vi "Register gRPC Methods.vi"(8 "error in (no error)":errorcluster, 11 "gRPC service in":refnum<class "CanWriterNixnet.lvclass">) -> (0 "error out":errorcluster, 3 "gRPC service out":refnum<class "CanWriterNixnet.lvclass">)   [LabVIEW 2021, in "CanWriterNixnet_server.lvlib" / "CanWriterNixnet.lvclass"]
uses:
  CanWriterNixnet.lvclass
  typeDefs/Server Internal UEs.ctl
  typeDefs/Server Internal Message.ctl
  typeDefs/Server gRPC UEs.ctl
  <vilib>/gRPC/LabVIEW gRPC Library/Server API/typeDefs/gRPCId Cluster.ctl
  <vilib>/gRPC/LabVIEW gRPC Library/Shared/grpcId.ctl
  CanWriterNixnet.lvclass/CanWriterNixnet.ctl
  <vilib>/gRPC/LabVIEW gRPC Library/grpc-lvsupport-release.lvlib
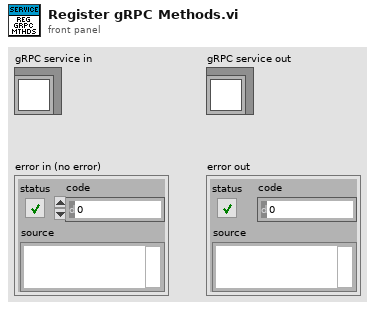
[diagram p1: front panel]
types:
  T1 = typedef "CanWriterNixnet_server.lvlib/CanWriterNixnet.lvclass/Server gRPC UEs.ctl" = cluster{"CanWriterNixnet GetDevices gRPC UE":refnum<user-event>, "CanWriterNixnet GetStatistics gRPC UE":refnum<user-event>, "CanWriterNixnet SetInterfaceBlink gRPC UE":refnum<user-event>, "CanWriterNixnet SendCanMessage gRPC UE":refnum<user-event>, "CanWriterNixnet GetCANStatus gRPC UE":refnum<user-event>}
  T2 = typedef "CanWriterNixnet_server.lvlib/CanWriterNixnet.lvclass/Server Internal UEs.ctl" = cluster{"CanWriterNixnet GetDevices Internal UE":refnum<user-event>, "CanWriterNixnet GetStatistics Internal UE":refnum<user-event>, "CanWriterNixnet SetInterfaceBlink Internal UE":refnum<user-event>, "CanWriterNixnet SendCanMessage Internal UE":refnum<user-event>, "CanWriterNixnet GetCANStatus Internal UE":refnum<user-event>}
  T3 = typedef "grpc-lvsupport-release.lvlib/grpcId.ctl" = u64
  T4 = typedef "CanWriterNixnet_server.lvlib/CanWriterNixnet.lvclass/Server Internal Message UE.ctl" = refnum<user-event>
  T5 = typedef "grpc-lvsupport-release.lvlib/gRPCId Cluster UE.ctl" = refnum<user-event>
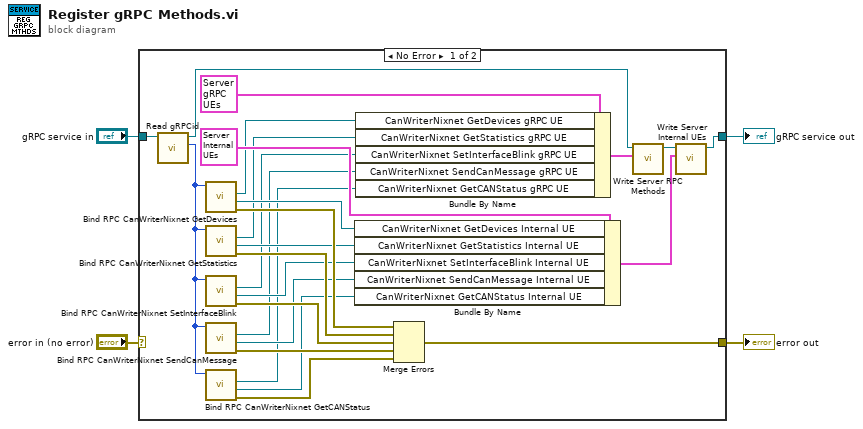
[diagram p0: block diagram]
diagram:
  n1 = case shown="No Error" "error in (no error)" {
    selector: "error in (no error)" -> [_ w30]
    tunnel: "gRPC service in" -> [w21 w31]
    tunnel: [w29 w30] -> w3
    tunnel: [w28 w31] -> w2
    frame No Error {
      n2 = call-dynamic "Read gRPCid.vi"("gRPC service in"=w21) -> ("gRPCid"=w20:T3, "gRPC service out"=w22:refnum<class "CanWriterNixnet.lvclass">)  [unwired: 8 in, 1 out]
      n3 = call "Bind RPC CanWriterNixnet GetDevices.vi"("gRPCid server in"=w20) -> ("error out"=w19:errorcluster, "CanWriterNixnet GetDevices Internal UE"=w17:T4, "CanWriterNixnet GetDevices gRPC UE"=w18:T5)  [unwired: 7 in, 1 out]
      n4 = call "Bind RPC CanWriterNixnet GetStatistics.vi"("gRPCid server in"=w20) -> ("error out"=w16:errorcluster, "CanWriterNixnet GetStatistics Internal UE"=w14:T4, "CanWriterNixnet GetStatistics gRPC UE"=w15:T5)  [unwired: 7 in, 1 out]
      n5 = call "Bind RPC CanWriterNixnet SetInterfaceBlink.vi"("gRPCid server in"=w20) -> ("error out"=w13:errorcluster, "CanWriterNixnet SetInterfaceBlink Internal UE"=w11:T4, "CanWriterNixnet SetInterfaceBlink gRPC UE"=w12:T5)  [unwired: 7 in, 1 out]
      n6 = call "Bind RPC CanWriterNixnet SendCanMessage.vi"("gRPCid server in"=w20) -> ("error out"=w10:errorcluster, "CanWriterNixnet SendCanMessage Internal UE"=w8:T4, "CanWriterNixnet SendCanMessage gRPC UE"=w9:T5)  [unwired: 7 in, 1 out]
      n7 = call "Bind RPC CanWriterNixnet GetCANStatus.vi"("gRPCid server in"=w20) -> ("error out"=w7:errorcluster, "CanWriterNixnet GetCANStatus Internal UE"=w5:T4, "CanWriterNixnet GetCANStatus gRPC UE"=w6:T5)  [unwired: 7 in, 1 out]
      n8 = Bundle By Name ("Bundle Internal UEs")(cluster=T2 {"CanWriterNixnet GetDevices Internal UE"=refnum, "CanWriterNixnet GetStatistics Internal UE"=refnum, "CanWriterNixnet SetInterfaceBlink Internal UE"=refnum, "CanWriterNixnet SendCanMessage Internal UE"=refnum, "CanWriterNixnet GetCANStatus Internal UE"=refnum} ("Server Internal UEs"), "CanWriterNixnet GetDevices Internal UE"=w17, "CanWriterNixnet GetStatistics Internal UE"=w14, "CanWriterNixnet SetInterfaceBlink Internal UE"=w11, "CanWriterNixnet SendCanMessage Internal UE"=w8, "CanWriterNixnet GetCANStatus Internal UE"=w5) -> (w27:T2)
      n9 = Bundle By Name ("Bundle gRPC UEs")(cluster=T1 {"CanWriterNixnet GetDevices gRPC UE"=refnum, "CanWriterNixnet GetStatistics gRPC UE"=refnum, "CanWriterNixnet SetInterfaceBlink gRPC UE"=refnum, "CanWriterNixnet SendCanMessage gRPC UE"=refnum, "CanWriterNixnet GetCANStatus gRPC UE"=refnum} ("gRPC Server Method Events"), "CanWriterNixnet GetDevices gRPC UE"=w18, "CanWriterNixnet GetStatistics gRPC UE"=w15, "CanWriterNixnet SetInterfaceBlink gRPC UE"=w12, "CanWriterNixnet SendCanMessage gRPC UE"=w9, "CanWriterNixnet GetCANStatus gRPC UE"=w6) -> (w24:T1)
      n10 = Merge Errors(w19, w16, w13, w10, w7) -> (w29:errorcluster)
      n11 = call "Write Server RPC Methods.vi"("Server RPC Methods"=w24, "gRPC service in"=w22) -> ("gRPC service out"=w25:refnum<class "CanWriterNixnet.lvclass">)  [unwired: 8 in, 1 out]
      n12 = call "Write Server Internal UEs.vi"("Server Internal UEs"=w27, "gRPC service in"=w25) -> ("gRPC service out"=w28:refnum<class "CanWriterNixnet.lvclass">)  [unwired: 8 in, 1 out]
    }
    frame Error {
    }
  }
  "error out" <- w3
  "gRPC service out" <- w2
